vi "Strip Error Details.vi"(8 "error in":errorcluster, 11 "text":string) -> (0 "error out":errorcluster, 3 "text out":string)   [LabVIEW 2020, in "MCP Server.lvlib"]
doc: "Removes what an MCP client must not see from an error text: the VI call chain (everything from the first -> to the end of the line), file paths (replaced by \"(path removed)\"), the tags <b>, </b>, <APPEND> and <ERR>, and line breaks. The remaining lines are joined with one space.\n\nUsed by Clean Error Message.vi."
uses:
  MCP Server.lvlib
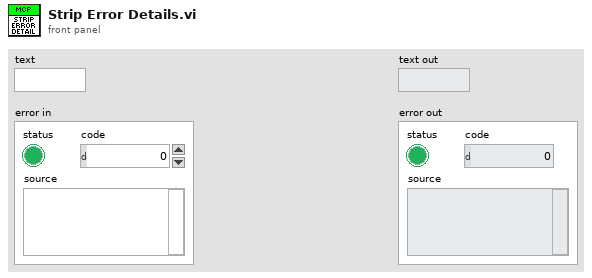
[diagram p1: front panel]
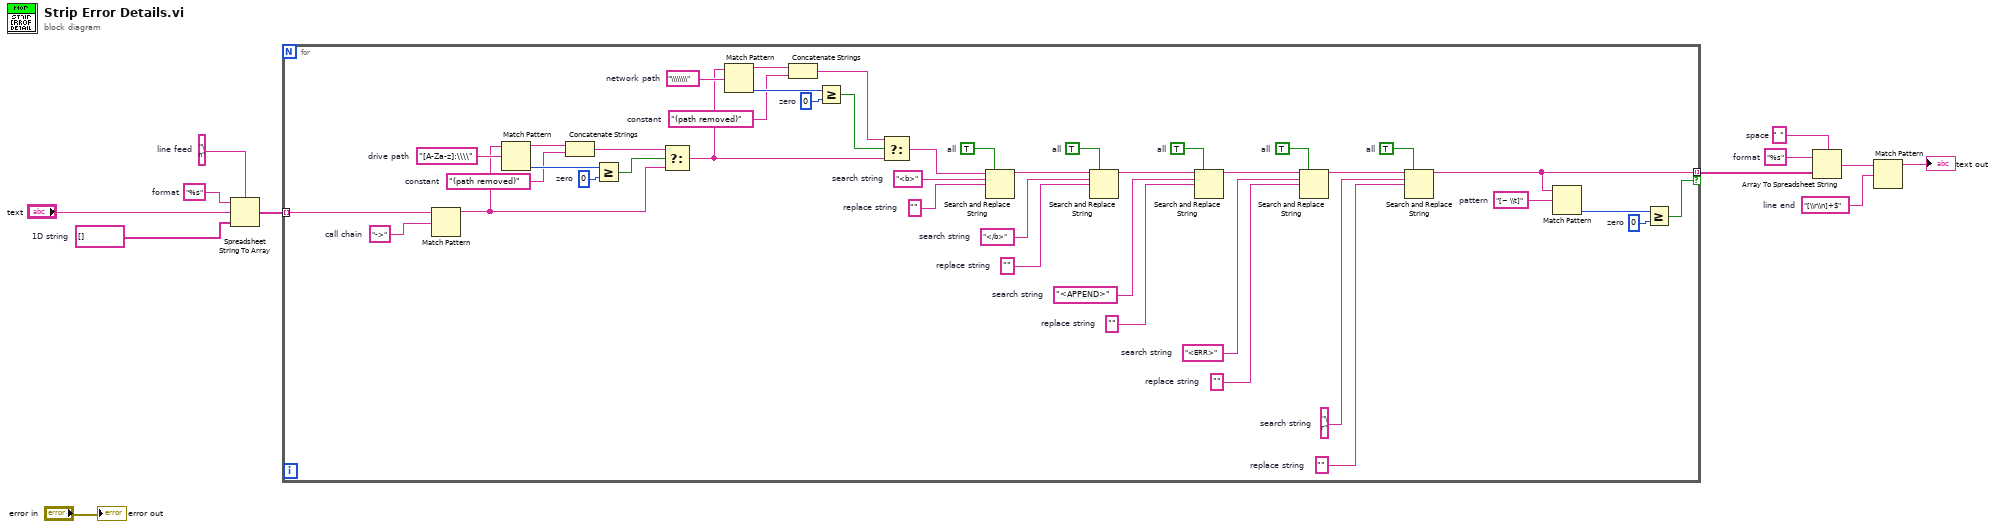
[diagram p0: block diagram]
diagram:
  w3 = "[\\r\\n]+$"  # line end
  w5 = " "  # space
  w7 = "%s"  # format
  w9 = "\n"  # line feed
  w10 = string[] []  # 1D string
  w12 = "%s"  # format
  n1 = Spreadsheet String To Array(delimiter (Tab)=w9, format string=w12, spreadsheet string="text", array type (2D Dbl)=w10) -> (array=w8:string[])
  n2 = for {
    tunnel: w8 -> [w55] mode=indexing
    tunnel: [w13] -> w6 mode=indexing if=w14
    w15 = 0  # zero
    w17 = "[~ \\t]"  # pattern
    w18 = TRUE  # all
    w19 = ""  # replace string
    w20 = "\r"  # search string
    w22 = TRUE  # all
    w23 = ""  # replace string
    w24 = "<ERR>"  # search string
    w26 = TRUE  # all
    w27 = ""  # replace string
    w28 = "<APPEND>"  # search string
    w30 = TRUE  # all
    w31 = ""  # replace string
    w32 = "</b>"  # search string
    w34 = TRUE  # all
    w35 = ""  # replace string
    w36 = "<b>"  # search string
    w41 = "(path removed)"  # constant
    w43 = 0  # zero
    w45 = "\\\\\\\\"  # network path
    w49 = "(path removed)"  # constant
    w51 = 0  # zero
    w53 = "[A-Za-z]:\\\\"  # drive path
    w54 = "->"  # call chain
    n3 = Match Pattern(string=w55, regular expression=w54) -> (before substring=w46:string)  [unwired: 1 in, 3 out]
    n4 = Match Pattern(string=w46, regular expression=w53) -> (before substring=w50:string, offset past match=w52:i32)  [unwired: 1 in, 2 out]
    n5 = Concatenate Strings(w50, w49) -> (w48:string)
    n6 = Greater Or Equal?(x=w52, y=w51) -> (x >= y?=w47:bool)
    n7 = Select(t=w48, s=w47, f=w46) -> (s? t:f=w38:string)
    n8 = Match Pattern(string=w38, regular expression=w45) -> (before substring=w42:string, offset past match=w44:i32)  [unwired: 1 in, 2 out]
    n9 = Concatenate Strings(w42, w41) -> (w40:string)
    n10 = Greater Or Equal?(x=w44, y=w43) -> (x >= y?=w39:bool)
    n11 = Select(t=w40, s=w39, f=w38) -> (s? t:f=w37:string)
    n12 = Search and Replace String(replace all?=w34, input string=w37, search string=w36, replace string=w35) -> (result string=w33:string)  [unwired: 4 in, 3 out]
    n13 = Search and Replace String(replace all?=w30, input string=w33, search string=w32, replace string=w31) -> (result string=w29:string)  [unwired: 4 in, 3 out]
    n14 = Search and Replace String(replace all?=w26, input string=w29, search string=w28, replace string=w27) -> (result string=w25:string)  [unwired: 4 in, 3 out]
    n15 = Search and Replace String(replace all?=w22, input string=w25, search string=w24, replace string=w23) -> (result string=w21:string)  [unwired: 4 in, 3 out]
    n16 = Search and Replace String(replace all?=w18, input string=w21, search string=w20, replace string=w19) -> (result string=w13:string)  [unwired: 4 in, 3 out]
    n17 = Match Pattern(string=w13, regular expression=w17) -> (offset past match=w16:i32)  [unwired: 1 in, 3 out]
    n18 = Greater Or Equal?(x=w16, y=w15) -> (x >= y?=w14:bool)
  }
  n19 = Array To Spreadsheet String(delimiter (Tab)=w5, array=w6, 3:w7) -> (spreadsheet string=w4:string)
  n20 = Match Pattern(string=w4, regular expression=w3) -> (before substring=→"text out":string)  [unwired: 1 in, 3 out]
  "error out" <- "error in"
